vi "Update Indicator Data.vi"(8 "formatted record":string, 9 "handler name":string, 10 "indicator data in":refnum<data-value>, 11 "registry in":T1[](array[typedef])) -> (2 "indicator data out":refnum<data-value>)   [LabVIEW 2018, in "GLog.lvlib" / "UI Updater.lvlib"]
uses:
  UI Updater.lvlib
  Handler Registration.ctl
  Indicator Data.ctl
panel:
  # "Connector Pane"
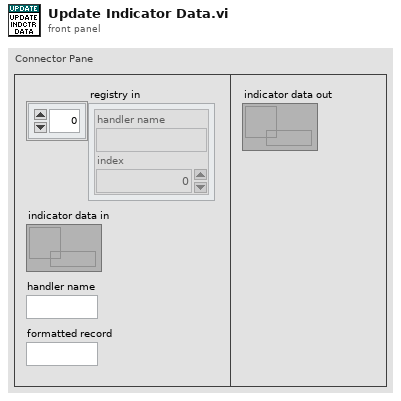
[diagram p1: front panel]
types:
  T1 = typedef "GLog.lvlib/UI Updater.lvlib/Handler Registration.ctl" = cluster{"handler name":string, "index":i32}
  T2 = typedef "GLog.lvlib/UI Updater.lvlib/Indicator Data.ctl" = cluster{"Ctl Ref":refnum<vi>, "Log Buffer":string[], "Log Limit":i32, "Line Limit":i32, "Autoscroll?":bool, "Valid?":bool, "Owning VI":refnum<vi>, "Ctl Index":i32, "Needs Write?":bool}
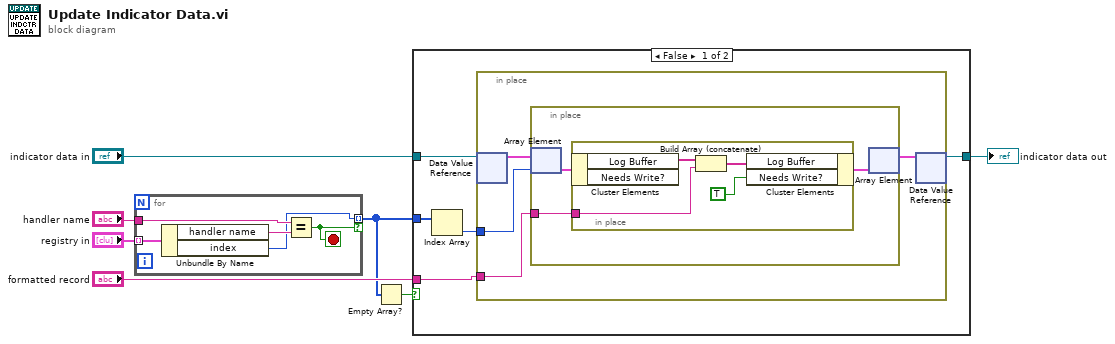
[diagram p0: block diagram]
diagram:
  n1 = for {
    tunnel: "registry in" -> [w8] mode=indexing
    tunnel: "handler name" -> [w12]
    tunnel: [w10] -> w3 mode=indexing if=w9
    stop <- w9 stop-if-true
    n2 = Unbundle By Name(w8) -> ("handler name"=w11:string, "index"=w10:i32)
    n3 = Equal?(x=w12, y=w11) -> (x = y?=w9:bool)
  }
  n4 = Empty Array?(array=w3) -> (empty?=w2:bool)
  n5 = case shown="False" w2 {
    tunnel: w3 -> [w17 _]
    tunnel: "indicator data in" -> [w16 w29]
    tunnel: "formatted record" -> [w14 _]
    tunnel: [w13 w29] -> w6
    frame False {
      n6 = Index Array(array=w17) -> (element=w15:i32)  [unwired: 1 in]
      n7 = in-place {
        in-place-border: w15 -> [w19]
        in-place-border: w14 -> [w21]
        n8 = in-place-dvr #1(w16) -> (w20:T2[])  [unwired: 1 out]
        n9 = in-place {
          in-place-border: w21 -> [w24]
          n10 = in-place-array #2(w20, w19) -> (w22:T2)
          n11 = in-place {
            in-place-border: w24 -> [w27]
            n12 = in-place-cluster #3(w22) -> ("Log Buffer"=w28:string[])  [unwired: 1 out]
            n13 = Build Array (concatenate)(w28, w27) -> (w26:string[])
            n14 = in-place-cluster #3("Log Buffer"=w26, "Needs Write?"=TRUE) -> (w23:T2)
          }
          n15 = in-place-array #2(w23) -> (w18:T2[])  [unwired: 1 out]
        }
        n16 = in-place-dvr #1(w18) -> (w13:refnum<data-value>)  [unwired: 1 out]
      }
    }
    frame True {
    }
  }
  "indicator data out" <- w6
